vi "Profile_Get_Next_Point.vi"(8 "error in (no error)":errorcluster={"status"=FALSE, "code"=0, "source"="\"\""}, 11 "ProfileContext and last result":string) -> (0 "error out":errorcluster={"status"=FALSE, "code"=0, "source"="\"\""}, 2 "status ok":bool, 3 "Next point or completed":string)   [LabVIEW 2026]
doc: "INTENT: Advance through operating points. LOGIC: Set per-point controller modes, target values, stabilization/dwell definitions."
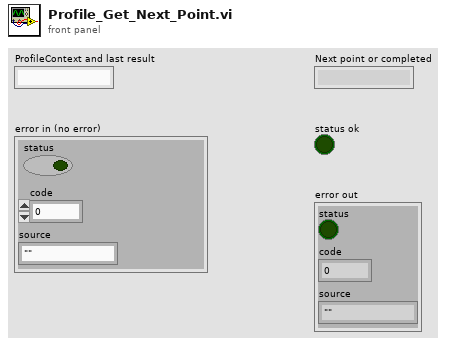
[diagram p1: front panel]
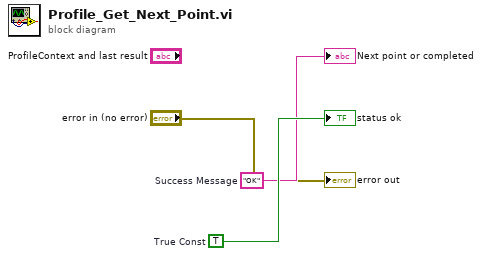
[diagram p0: block diagram]
diagram:
  w3 = TRUE  # True Const
  w2 = "OK"  # Success Message
  "Next point or completed" <- w2
  "status ok" <- w3
  "error out" <- "error in (no error)"
